vi "Connect.vi"(8 "error in (no error)":errorcluster, 10 "Connection String":string, 11 "PostgresqlConnection in":refnum<class "DBC.lvclass">) -> (0 "error out":errorcluster, 3 "PostgresqlConnection out":refnum<class "DBC.lvclass">)   [LabVIEW 2026, in "ORM_DBC_Npgsql_netCore.lvlib" / "DBC.lvclass"]
uses:
  DBC.lvclass
  <vilib>/Viviota/shared/data_nc/Npgsql.dll
  <vilib>/Viviota/shared/ORM_DBC_dotNetCore.lvlibp/Write connection.vi
  <vilib>/Viviota/shared/ORM.lvlibp/DbConnection/Write ColumnNameEqualsValueFormat.vi
  <vilib>/Viviota/shared/ORM.lvlibp/DbConnection/Write ColumnNameFormat.vi
  <vilib>/Viviota/shared/ORM.lvlibp/DbConnection/Write LastIdentityQuery.vi
  <vilib>/Viviota/shared/ORM.lvlibp/DbConnection/Write SupportBulkCreate.vi
  DBC.lvclass/DBC.ctl
panel:
  # "Server=localhost;Port=5432;Database=testdb;User Id=postgres;\nPassword=password;"
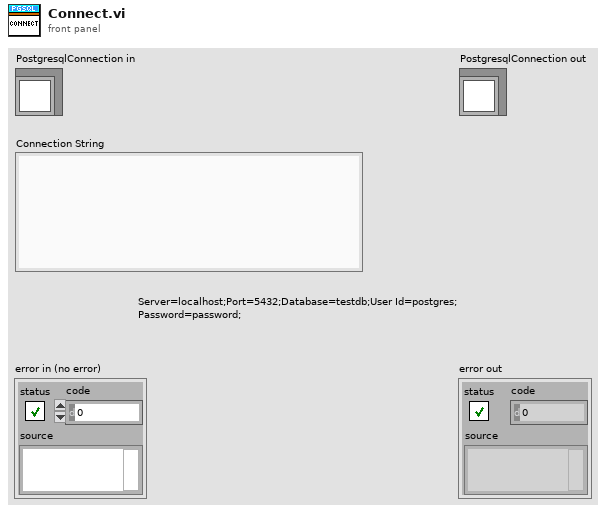
[diagram p1: front panel]
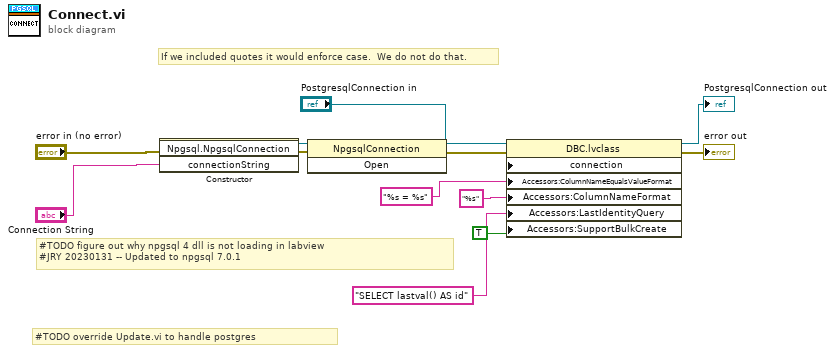
[diagram p0: block diagram]
diagram:
  # "If we included quotes it would enforce case.  We do not do that."
  # "#TODO override Update.vi to handle postgres"
  # "#TODO figure out why npgsql 4 dll is not loading in labview\n#JRY 20230131 -- Updated to npgsql 7.0.1"
  n1 = constructor class="NpgsqlConnection"(error in="error in (no error)", "connectionString"="Connection String") -> (reference out=w8:refnum<k39>, error out=w4:errorcluster)  [unwired: 2 in, 2 out]
  n2 = invoke class="NpgsqlConnection" method="Open"(reference=w8, error in=w4) -> (reference out=w5:refnum<k39>, error out=w7:errorcluster)  [unwired: 1 in, 1 out]
  n3 = property class="DBC.lvclass"(reference="PostgresqlConnection in", error in=w7, "connection"=w5, "Accessors:ColumnNameEqualsValueFormat"="%s = %s" ("ColumnNameFormat"), "Accessors:ColumnNameFormat"="%s" ("ColumnNameFormat"), "Accessors:LastIdentityQuery"="SELECT lastval() AS id" ("LastIdentityQuery"), "Accessors:SupportBulkCreate"=TRUE ("SupportBulkCreate")) -> (reference out=→"PostgresqlConnection out":refnum<class "DBC.lvclass">, error out=→"error out":errorcluster)
